vi "Set Message Field Representation.vi"(8 "error in (no error)":errorcluster, 10 "MessageElementType":T1, 11 "Control ref in":refnum<vi>) -> (0 "error out":errorcluster, 3 "Control ref out":refnum<vi>)   [LabVIEW 2019, in "gRPC Template Creation Utility.lvlib"]
uses:
  gRPC Template Creation Utility.lvlib
  TypeDefs/Message Element Type.ctl
  <vilib>/numeric/LVNumericRepresentation.ctl
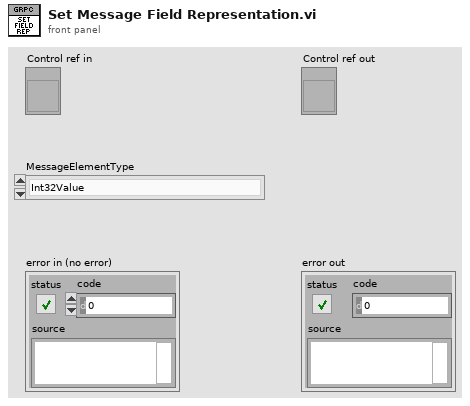
[diagram p1: front panel]
types:
  T1 = typedef "gRPC Template Creation Utility.lvlib/Message Element Type.ctl" = enum32{"Int32Value", "FloatValue", "DoubleValue", "BoolValue", "StringValue", "MessageValue", "Int64Value", "UInt32Value", "UInt64Value", "EnumValue", "Bytes", "Fixed64", "Fixed32", "SFixed64", "SFixed32", "SInt64", "SInt32"}
  T2 = typedef "LVNumericRepresentation.ctl" = enum32{"Extended Precision", "Double Precision", "Single Precision", "Long", "Word", "Byte", "Unsigned Long", "Unsigned Word", "Unsigned Byte", "Complex Extended", "Complex Double", "Complex Single", "Quad", "Unsigned Quad", "Fixed-Point"}
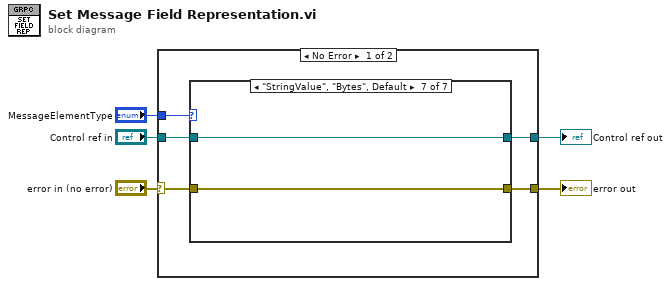
[diagram p0: block diagram]
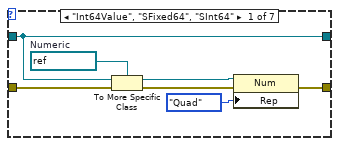
[diagram p2: hidden frame]
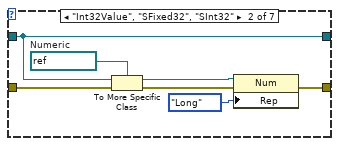
[diagram p3: hidden frame]
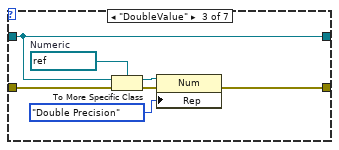
[diagram p4: hidden frame]
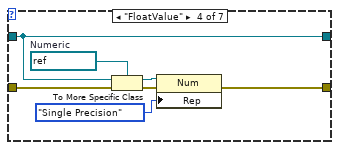
[diagram p5: hidden frame]
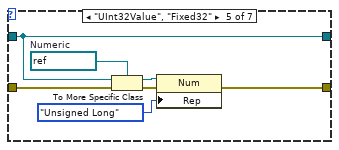
[diagram p6: hidden frame]
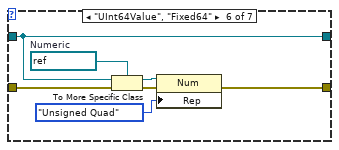
[diagram p7: hidden frame]
diagram:
  n1 = case shown="No Error" "error in (no error)" {
    selector: "error in (no error)" -> [w6 w55]
    tunnel: [w10 w56] -> w5
    tunnel: "MessageElementType" -> [w9 _]
    tunnel: [w8 w55] -> w3
    tunnel: "Control ref in" -> [w7 w56]
    frame No Error {
      n2 = case shown="\"StringValue\", \"Bytes\", Default" w9 {
        tunnel: w7 -> [w11 w18 w25 w32 w39 w46 w54]
        tunnel: w6 -> [w13 w23 w30 w37 w41 w48 w53]
        tunnel: [w12 w19 w26 w33 w40 w47 w53] -> w8
        tunnel: [w11 w18 w25 w32 w39 w46 w54] -> w10
        frame "Int64Value", "SFixed64", "SInt64" {
          w17 = refnum<vi> refnum  # Numeric
          n3 = To More Specific Class(target class=w17, reference=w11, error in=w13) -> (specific class reference=w16:refnum<vi>, error out=w15:errorcluster)
          n4 = property class="Num"(reference=w16, error in=w15, "Rep"=LVNumericRepresentation."Quad" ("Representation")) -> (error out=w12:errorcluster)  [unwired: 1 out]
        }
        frame "Int32Value", "SFixed32", "SInt32" {
          w24 = refnum<vi> refnum  # Numeric
          n5 = To More Specific Class(target class=w24, reference=w18, error in=w23) -> (specific class reference=w22:refnum<vi>, error out=w21:errorcluster)
          n6 = property class="Num"(reference=w22, error in=w21, "Rep"=LVNumericRepresentation."Long" ("Representation")) -> (error out=w19:errorcluster)  [unwired: 1 out]
        }
        frame "DoubleValue" {
          w31 = refnum<vi> refnum  # Numeric
          n7 = To More Specific Class(target class=w31, reference=w25, error in=w30) -> (specific class reference=w29:refnum<vi>, error out=w28:errorcluster)
          n8 = property class="Num"(reference=w29, error in=w28, "Rep"=LVNumericRepresentation."Double Precision" ("Representation")) -> (error out=w26:errorcluster)  [unwired: 1 out]
        }
        frame "FloatValue" {
          w38 = refnum<vi> refnum  # Numeric
          n9 = To More Specific Class(target class=w38, reference=w32, error in=w37) -> (specific class reference=w36:refnum<vi>, error out=w35:errorcluster)
          n10 = property class="Num"(reference=w36, error in=w35, "Rep"=LVNumericRepresentation."Single Precision" ("Representation")) -> (error out=w33:errorcluster)  [unwired: 1 out]
        }
        frame "UInt32Value", "Fixed32" {
          w45 = refnum<vi> refnum  # Numeric
          n11 = To More Specific Class(target class=w45, reference=w39, error in=w41) -> (specific class reference=w44:refnum<vi>, error out=w43:errorcluster)
          n12 = property class="Num"(reference=w44, error in=w43, "Rep"=LVNumericRepresentation."Unsigned Long" ("Representation")) -> (error out=w40:errorcluster)  [unwired: 1 out]
        }
        frame "UInt64Value", "Fixed64" {
          w52 = refnum<vi> refnum  # Numeric
          n13 = To More Specific Class(target class=w52, reference=w46, error in=w48) -> (specific class reference=w51:refnum<vi>, error out=w50:errorcluster)
          n14 = property class="Num"(reference=w51, error in=w50, "Rep"=LVNumericRepresentation."Unsigned Quad" ("Representation")) -> (error out=w47:errorcluster)  [unwired: 1 out]
        }
        frame "StringValue", "Bytes", Default {
        }
      }
    }
    frame Error {
    }
  }
  "Control ref out" <- w5
  "error out" <- w3
